vi "set Measurement Window Mode - FSV40.vi"(8 "error in (no error)":errorcluster, 10 "Measurement Window Mode":T1, 11 "Keysight 9020A in":refnum<class "Keysight 9020A.lvclass">) -> (0 "error out":errorcluster, 3 "Keysight 9020A out":refnum<class "Keysight 9020A.lvclass">)   [LabVIEW 2023, in "Spectrum Analyzer.lvlib" / "Keysight 9020A.lvclass"]
doc: "1) ACPower\nAdjacent-channel power measurement with a single carrier signal\n2) CPOWer\nChannel power measurement with a single carrier signal (equivalent to adjacent-channel power measurement with \"NO. OF ADJ CHAN\" = 0)\n3) MCACpower\nChannel/adjacent-channel power measurement with several carrier signals\n4) OBANdwidth | OBWidth\nMeasurement of occupied bandwidth\n5) CN\nMeasurement of carrier-to-noise ratio\n6) CN0\nMeasurement of carrier-to-noise ratio referenced to 1 Hz bandwidth"
uses:
  Keysight 9020A.lvclass
  TYPE DEFINITION/TYPE Measurement Window Mode.ctl
  Keysight 9020A.lvclass/Keysight 9020A.ctl
  Spectrum Analyzer.lvlib
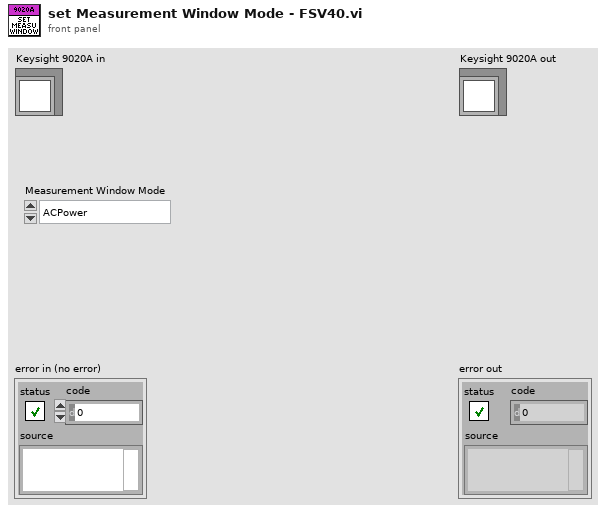
[diagram p1: front panel]
types:
  T1 = typedef "Spectrum Analyzer.lvlib/TYPE Measurement Window Mode.ctl" = enum16{"ACPower", "CPOWer", "MCACpower", "OBANdwidth", "OBWidth", "CN", "CN0"}
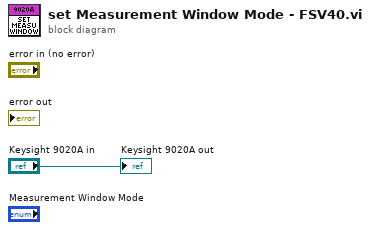
[diagram p0: block diagram]
diagram:
  "Keysight 9020A out" <- "Keysight 9020A in"
